vi "ZM-CM-createResources.vi"(8 "error in (no error)":errorcluster, 11 "ZM-CM-communication_manager in":refnum<class "ZM-CM-communication_manager.lvclass">) -> (0 "error out":errorcluster, 3 "ZM-CM-communication_manager out":refnum<class "ZM-CM-communication_manager.lvclass">)   [LabVIEW 2020, in "ZM-CM-communication_manager.lvlib" / "ZM-CM-communication_manager.lvclass"]
doc: "Creates the communication manager's resources in Pre Launch Init: initialises the protocol from the pre-launch settings (ZM-CP-init: the file logger creates its folder, the UDP sender opens its socket) and stores it. If init fails, it releases the protocol and returns the original error, so the launch fails."
uses:
  ZM-CM-communication_manager.lvclass
  ZM-CM-communication_manager.lvclass/ZM-CM-communication_manager.ctl
  protocol/ZM-CP-communication_protocol/ZM-CP-communication_protocol/ZM-CP-communication_protocol.lvclass
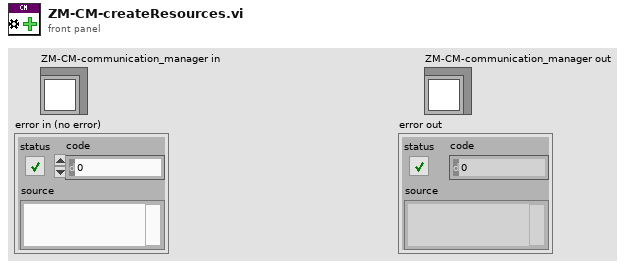
[diagram p1: front panel]
types:
  T1 = typedef "ZM-CM-communication_manager.lvlib/ZM-CM-communication_manager.lvclass/ZM-CM-PRELAUNCH_SETTINGS.ctl" = cluster{"protocol":refnum<class "ZM-CP-communication_protocol.lvclass">}
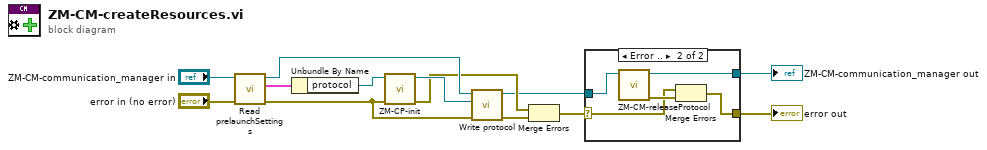
[diagram p0: block diagram]
diagram:
  n1 = call "Read prelaunchSettings.vi"("error in (no error)"="error in (no error)", "ZM-CM-communication_manager in"="ZM-CM-communication_manager in") -> ("error out"=w9:errorcluster, "ZM-CM-PRELAUNCH_SETTINGS"=w11:T1, "ZM-CM-communication_manager out"=w8:refnum<class "ZM-CM-communication_manager.lvclass">)  [unwired: 7 in]
  n2 = Unbundle By Name(w11) -> ("protocol"=w10:refnum<class "ZM-CP-communication_protocol.lvclass">)
  n3 = call-dynamic "ZM-CP-init.vi"("error in (no error)"=w9, "ZM-CP-communication_protocol in"=w10) -> ("error out"=w6:errorcluster, "ZM-CP-communication_protocol out"=w7:refnum<class "ZM-CP-communication_protocol.lvclass">)  [unwired: 8 in]
  n4 = call "Write protocol.vi"("error in (no error)"=w9, "ZM-CP-communication_protocol.lvlib:ZM-CP-communication_protocol.lvclass"=w7, "ZM-CM-communication_manager in"=w8) -> ("error out"=w5:errorcluster, "ZM-CM-communication_manager out"=w4:refnum<class "ZM-CM-communication_manager.lvclass">)  [unwired: 7 in]
  n5 = Merge Errors(w6, w5) -> (w3:errorcluster)
  n6 = case shown="Error .." w3 {
    selector: w3 -> [w14 w16]
    tunnel: w4 -> [w15 w20]
    tunnel: [w15 w18] -> w2
    tunnel: [w14 w17] -> w1
    frame No Error {
    }
    frame Error {
      n7 = call "ZM-CM-releaseProtocol.vi"("ZM-CM-communication_manager in"=w20) -> ("error out"=w19:errorcluster, "ZM-CM-communication_manager out"=w18:refnum<class "ZM-CM-communication_manager.lvclass">)  [unwired: 9 in]
      n8 = Merge Errors(w16, w19) -> (w17:errorcluster)
    }
  }
  "ZM-CM-communication_manager out" <- w2
  "error out" <- w1
